vi "ot-hold-last-values-test.vi"(8 "error in (no error)":errorcluster) -> (0 "error out":errorcluster, 2 "Held Length":i32[](array[numeric]), 3 "Held Values":dbl[][](array[numeric]))   [LabVIEW 2026]
doc: "Unit test for OT Hold Last Values.vi: one call per row of the call sequence (new values, update?, reset?, reset values). Returns the held values of every call (numeric only)."
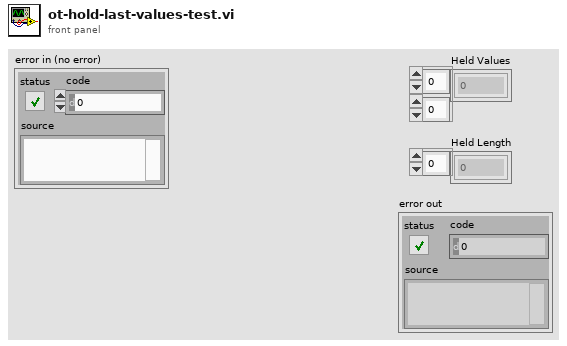
[diagram p1: front panel]
types:
  T1 = cluster{"new values":dbl[], "update?":bool, "reset?":bool, "reset values":dbl[]}[]
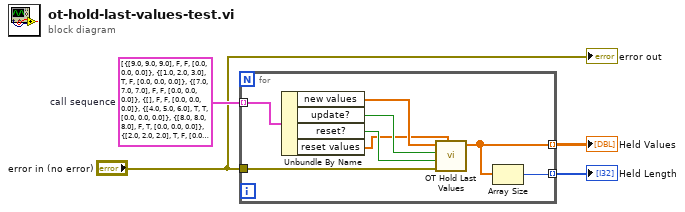
[diagram p0: block diagram]
diagram:
  w4 = T1 [{"new values"=[9.0, 9.0, 9.0], "update?"=FALSE, "reset?"=FALSE, "reset values"=[0.0, 0.0, 0.0]}, {"new values"=[1.0, 2.0, 3.0], "update?"=TRUE, "reset?"=FALSE, "reset values"=[0.0, 0.0, 0.0]}, {"new values"=[7.0, 7.0, 7.0], "update?"=FALSE, "reset?"=FALSE, "reset values"=[0.0, 0.0, 0.0]}, {"new values"=[], "update?"=FALSE, "reset?"=FALSE, "reset values"=[0.0, 0.0, 0.0]}, {"new values"=[4.0, 5.0, 6.0], "update?"=TRUE, "reset?"=TRUE, "reset values"=[0.0, 0.0, 0.0]}, {"new values"=[8.0, 8.0, 8.0], "update?"=FALSE, "reset?"=TRUE, "reset values"=[0.0, 0.0, 0.0]}, {"new values"=[2.0, 2.0, 2.0], "update?"=TRUE, "reset?"=FALSE, "reset values"=[0.0, 0.0, 0.0]}, {"new values"=[1.0, 1.0], "update?"=FALSE, "reset?"=FALSE, "reset values"=[0.0, 0.0]}]  # call sequence
  n1 = for {
    tunnel: w4 -> [w12] mode=indexing
    tunnel: "error in (no error)" -> [w7]
    tunnel: [w6] -> w3 mode=indexing
    tunnel: [w5] -> w2 mode=indexing
    n2 = Unbundle By Name(w12) -> ("new values"=w11:dbl[], "update?"=w10:bool, "reset?"=w9:bool, "reset values"=w8:dbl[])
    n3 = call "OT Hold Last Values.vi"("reset values"=w8, "error in (no error)"=w7, "reset? (F)"=w9, "update?"=w10, "new values"=w11) -> ("held values"=w6:dbl[])  [unwired: 5 in, 1 out]
    n4 = Array Size(array=w6) -> (size(s)=w5:i32)
  }
  "Held Values" <- w3
  "Held Length" <- w2
  "error out" <- "error in (no error)"
